vi "Process.vi"(8 "error in":errorcluster, 11 "Qbus in":refnum<class "Qbus.lvclass">) -> (0 "error out":errorcluster)   [LabVIEW 2021, in "AnalogGenerationProcess.lvlib"]
uses:
  AnalogGenerationProcess.lvlib
  <vilib>/addons/Qbus/Qbus.lvclass
  controls/state.ctl
  controls/generation status.ctl
  <vilib>/addons/_NISVFA/_Generation/Signal Generation/SV Signal/SV Signal.lvclass
  controls/analog generation settings.ctl
  controls/analog output settings.ctl
  controls/terminal configuration.ctl
  controls/signal settings.ctl
  controls/signal type.ctl
  shared/controls/digital output level units.ctl
  controls/sine wave properties.ctl
  <vilib>/addons/_NISVFA/_Generation/Signal Generation/SV Signal/sv_System Timing Model.ctl
  <vilib>/DAQmx/write.llb/DAQmx Write (Analog 1D Wfm NChan NSamp).vi
  <vilib>/addons/_NISVFA/_Generation/Signal Generation/SV Sinusoid/SV Sinusoid.lvclass
  C:/Program Files/National Instruments/LabVIEW 2021/vi.lib/addons/_NISVFA/_Generation/Signal Generation/SV Signal/SV Signal.lvclass
  <vilib>/addons/_NISVFA/_Generation/Signal Generation/SV Sinusoid/Configure Sine.vi
  <vilib>/addons/_NISVFA/_Generation/Signal Generation/SV Signal/Write Sample Rate.vi
  <vilib>/addons/_NISVFA/_Generation/Signal Generation/SV Signal/Write System Timing Model.vi
  <vilib>/addons/_NISVFA/_Generation/Signal Generation/SV Signal/Write Ramp Parameters.vi
  <vilib>/DAQmx/miscellaneous.llb/DAQmx Fill In Error Info.vi
  subVIs/utility/AudioGenUtility.lvlib
  shared/logger process/EventLoggerProcess.lvlib
  controls/AudioGenTypeDefs.lvlib
  shared/controls/audio controls.lvlib
  C:/Program Files/National Instruments/LabVIEW 2021/vi.lib/addons/_NISVFA/_Generation/Signal Generation/SV Function/SV Function.lvclass
  C:/Program Files/National Instruments/LabVIEW 2021/vi.lib/addons/_NISVFA/_Generation/Signal Generation/SV Sinusoid/SV Sinusoid.lvclass
  <vilib>/addons/_NISVFA/_Generation/Signal Generation/SV Multitone/SV Multitone.lvclass
  C:/Program Files/National Instruments/LabVIEW 2021/vi.lib/addons/_NISVFA/_Generation/Signal Generation/SV Multitone/SV Multitone.lvclass
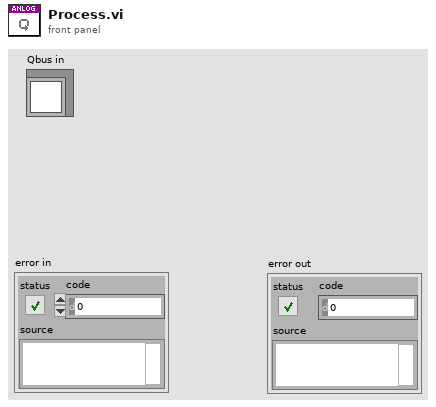
[diagram p1: front panel]
types:
  T1 = typedef "AnalogGenerationProcess.lvlib/state.ctl" = cluster{"DAQmx task":refnum<k21>, "status":T2, "signals":refnum<class "SV Signal.lvclass">[], "number of channels":u32}
  T2 = typedef "AudioGenTypeDefs.lvlib/generation status.ctl" = enum16{"Idle", "Committed", "Active"}
  T3 = typedef "AudioGenTypeDefs.lvlib/analog generation settings.ctl" = cluster{"channel list":string, "output settings":T4, "signal settings":T6}
  T4 = typedef "AudioGenTypeDefs.lvlib/analog output settings.ctl" = cluster{"output rate":dbl, "range":dbl, "terminal configuration":T5, "output impedance":dbl, "common mode offset":dbl, "pure tone mode":bool}
  T5 = typedef "AudioGenTypeDefs.lvlib/terminal configuration.ctl" = enum32{"Default", "RSE", "Differential", "Pseudodifferential"}
  T6 = typedef "AudioGenTypeDefs.lvlib/signal settings.ctl" = cluster{"signal type":T7, "properties":string, "output level units":T8}
  T7 = typedef "AudioGenTypeDefs.lvlib/signal type.ctl" = enum16{"Sine", "Dual Tone"}
  T8 = typedef "audio controls.lvlib/digital output level units.ctl" = enum32{"% FS", "dBFS", "V"}
  T9 = cluster{"profile":enum16{"Linear", "Half cosine"}, "durations [s]":cluster{"ramp-up":dbl, "transition":dbl, "ramp-down":dbl}}
  T10 = typedef "AudioGenTypeDefs.lvlib/sine wave properties.ctl" = cluster{"frequency":dbl, "amplitude":dbl, "phase":dbl}[]
  T11 = typedef "AudioGenTypeDefs.lvlib/dual tone properties.ctl" = cluster{"IMD type":T12, "low frequency":dbl, "high frequency":dbl, "amplitude ratio":dbl, "ampltidue":dbl}
  T12 = typedef "AudioGenTypeDefs.lvlib/dual tone types.ctl" = enum32{"SMPTE 4:1", "DIN", "CCIF 11k-12k", "CCIF 19k-20k", "Custom"}
  T13 = typedef "SV Signal.lvclass/sv_System Timing Model.ctl" = i64
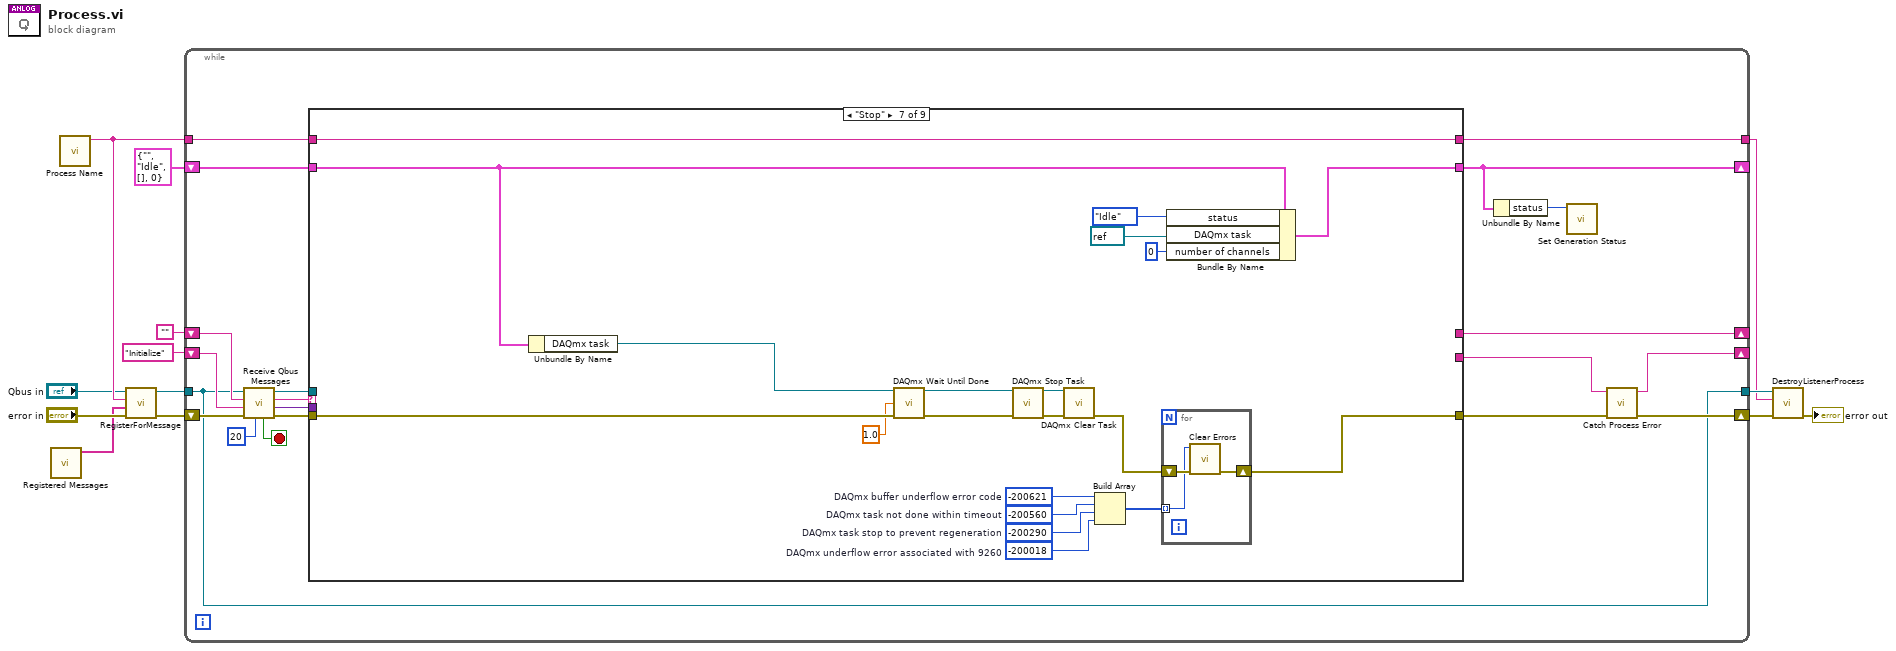
[diagram p0: block diagram]
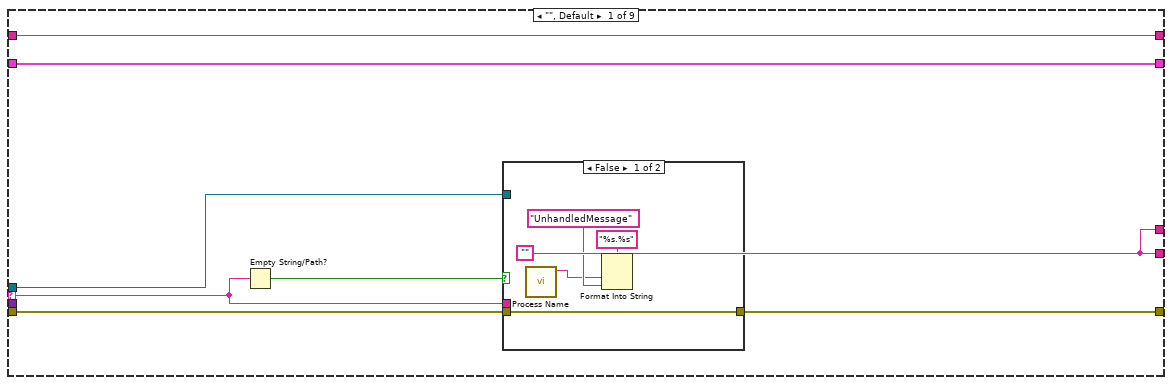
[diagram p2: hidden frame]
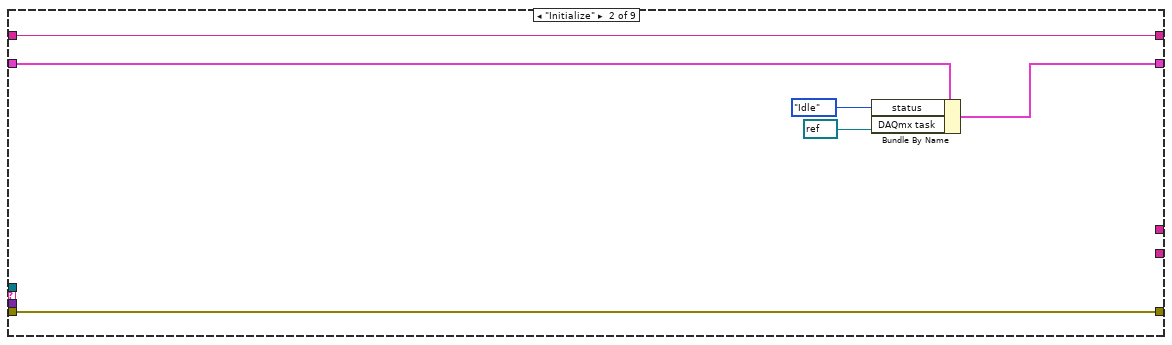
[diagram p4: hidden frame]
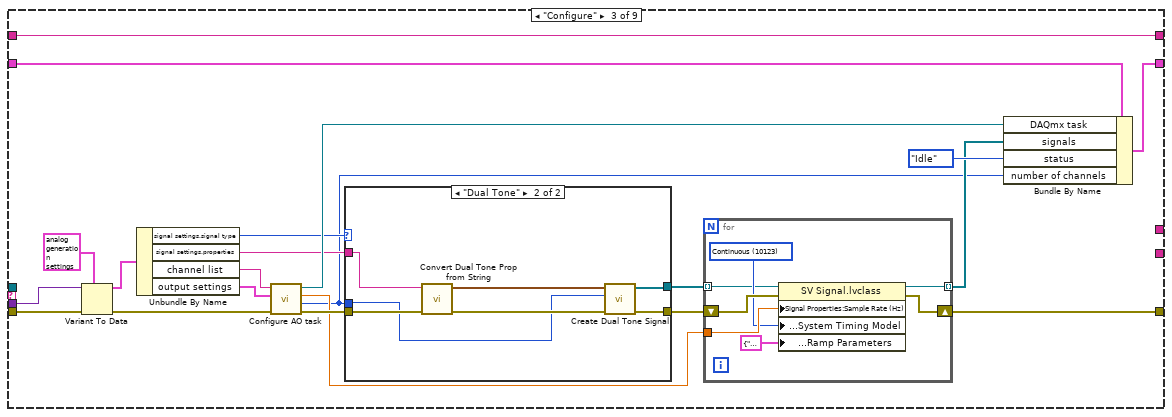
[diagram p5: hidden frame]
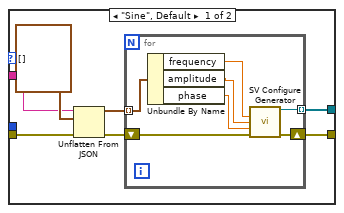
[diagram p6: hidden frame]
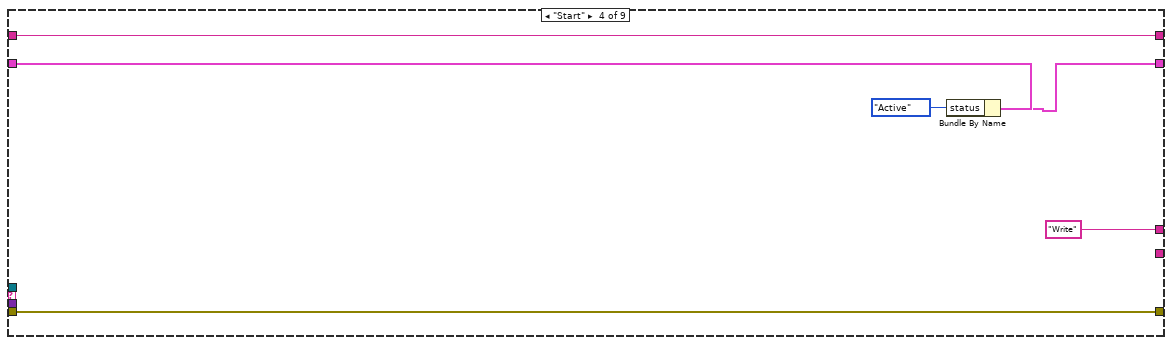
[diagram p7: hidden frame]
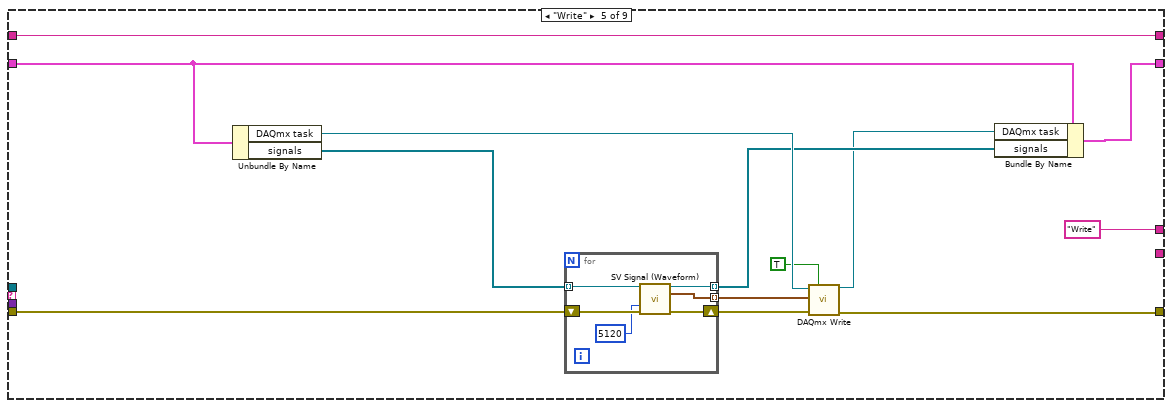
[diagram p8: hidden frame]
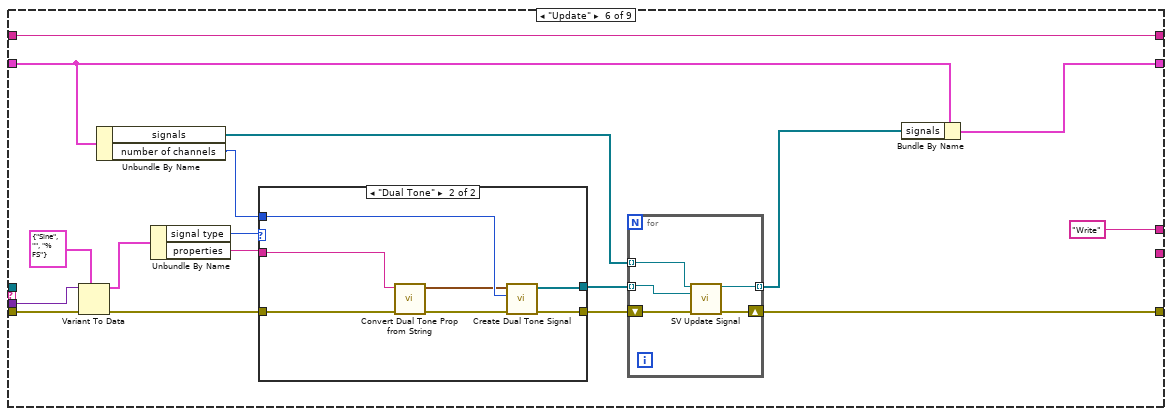
[diagram p9: hidden frame]
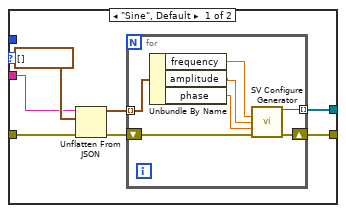
[diagram p10: hidden frame]
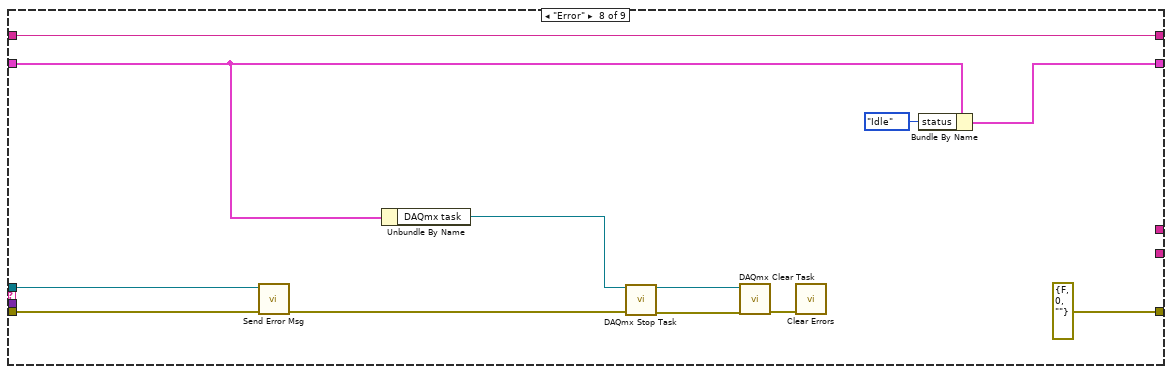
[diagram p11: hidden frame]
diagram:
  n1 = call "Registered Messages.vi"() -> ("registered messages"=w6:string[])  [unwired: 11 in]
  n2 = call "Process Name.vi"() -> ("process name"=w9:string)  [unwired: 11 in]
  n3 = call <vilib>:"RegisterForMessage.vi"("error in (no error)"="error in", "message names"=w6, "process name"=w9, "Qbus in"="Qbus in") -> ("error in (no error)"=w12:errorcluster, "Qbus out"=w13:refnum<class "Qbus.lvclass">)  [unwired: 6 in]
  n4 = while {
    shift-right: [w20] -> _
    shift-left: "" -> [w32]
    tunnel: w13 -> [w16]
    tunnel: w9 -> [w18]
    tunnel: [w16] -> w4
    tunnel: [w22] -> w2
    shift-right: [w26] -> _
    shift-left: "Initialize" -> [w28]
    shift-right: [w27] -> w5
    shift-left: w12 -> [w25]
    shift-right: [w15] -> _
    shift-left: T1 {"DAQmx task"="", "status"=enum."Idle", "signals"=[], "number of channels"=0} ("state") -> [w17]
    stop <- w33 stop-if-true
    n5 = call "Receive Qbus Messages.vi"("timeout(ms)"=20 ("milliseconds to wait"), "error in (no error)"=w25, "priority action"=w28, "default action"=w32, "Qbus in"=w16) -> ("error out"=w31:errorcluster, "message value"=w29:variant, "action"=w24:string, "Qbus out"=w30:refnum<class "Qbus.lvclass">, "exit"=w33:bool)  [unwired: 2 in]
    n6 = case shown="\"Stop\"" w24 {
      selector: w24 -> [w38 _ _ _ _ _ _ _ _]
      tunnel: w31 -> [w40 w52 w64 w107 w119 w139 w188 w203 w207]
      tunnel: w30 -> [w36 _ _ _ _ _ _ w202 _]
      tunnel: [w39 w52 w68 w107 w115 w129 w176 errorcluster {"status"=FALSE, "code"=0, "source"=""} ("error out") w207] -> w19
      tunnel: w29 -> [_ _ w65 _ _ w138 _ _ _]
      tunnel: [w41 w51 w73 w106 w120 w143 w189 w204 w206] -> w22
      tunnel: w18 -> [w41 w51 w73 w106 w120 w143 w189 w204 w206]
      tunnel: [w35 _ _ _ _ _ _ _ _] -> w21
      tunnel: [w35 _ _ "Write" "Write" "Write" _ _ _] -> w20
      tunnel: w17 -> [w34 w50 w72 w105 w111 w142 w184 w195 w205]
      tunnel: [w34 w49 w71 w103 w110 w141 w183 w194 w205] -> w15
      frame "", Default {
        w35 = ""
        n7 = Empty String/Path?(string/path=w38) -> (empty?=w37:bool)
        n8 = case shown="False" w37 {
          tunnel: [w42 w46] -> w39
          tunnel: w40 -> [w42 w46]
          tunnel: w38 -> [_ _]
          tunnel: w36 -> [_ _]
          frame False {
            n9 = call "Process Name.vi"() -> ("process name"=w43:string)  [unwired: 11 in]
            n10 = Format Into String(format string="%s.%s", w43, "UnhandledMessage" ("ProcessName")) -> ()  [unwired: 2 in, 2 out]
          }
          frame True {
          }
        }
      }
      frame "Initialize" {
        n11 = Bundle By Name(cluster=w50, "status"=enum16{"Idle", "Committed", "Active"}."Idle", "DAQmx task"=refnum<k21> refnum) -> (w49:T1)
      }
      frame "Configure" {
        n12 = Variant To Data(error in=w64, type=T3 {"channel list"="", "output settings"={"output rate"=0.0, "range"=0.0, "terminal configuration"=enum."Pseudodifferential", "output impedance"=0.0, "common mode offset"=0.0, "pure tone mode"=FALSE}, "signal settings"={"signal type"=enum."Sine", "properties"="", "output level units"=enum."% FS"}} ("analog generation"), Variant=w65) -> (data=w62:T3, error out=w61:errorcluster)
        n13 = Unbundle By Name(w62) -> ("signal settings.signal type"=w60:T7, "signal settings.properties"=w59:string, "channel list"=w58:string, "output settings"=w57:T4)
        n14 = call "Configure AO task.vi"("error in (no error)"=w61, "analog generation"=w57, "physical channels"=w58) -> ("error out"=w70:errorcluster, "number of channels"=w53:u32, "actual sample rate"=w67:dbl, "task out"=w66:refnum<k21>)  [unwired: 5 in]
        n15 = case shown="\"Dual Tone\"" w60 {
          tunnel: w70 -> [w85 w101]
          tunnel: [w87 w96] -> w55
          tunnel: [w86 w99] -> w69
          tunnel: w59 -> [w82 w100]
          tunnel: w53 -> [_ w95]
          frame "Sine", Default {
            n16 = Unflatten From JSON(JSON string=w82, type and defaults=T10 [] ("sine wave properties"), error in (no error)=w85) -> (value=w81:T10, error out=w84:errorcluster)  [unwired: 4 in]
            n17 = for {
              tunnel: [w94] -> w87 mode=indexing
              shift-right: [w93] -> w86
              shift-left: w84 -> [w92]
              tunnel: w81 -> [w91] mode=indexing
              n18 = Unbundle By Name(w91) -> ("frequency"=w90:dbl, "amplitude"=w89:dbl, "phase"=w88:dbl)
              n19 = call-poly <vilib>:"SV Configure Generator.vi"("frequency (Hz)"=w90, "amplitude"=w89, "phase (deg)"=w88, "error in (no error)"=w92) -> ("signal configuration"=w94:refnum<class "SV Sinusoid.lvclass">, "error out"=w93:errorcluster)  [unwired: 10 in]
            }
          }
          frame "Dual Tone" {
            n20 = call "Convert Dual Tone Prop from String.vi"("error in (no error)"=w101, "dual tone properties"=w100) -> ("error out"=w98:errorcluster, "dual tone properties"=w97:T11)  [unwired: 8 in]
            n21 = call "Create Dual Tone Signal.vi"("error in (no error)"=w98, "number of channels"=w95, "dual tone properties"=w97) -> ("error out"=w99:errorcluster, "signals"=w96:refnum<class "SV Multitone.lvclass">[])  [unwired: 7 in]
          }
        }
        n22 = for {
          tunnel: w67 -> [w78]
          shift-right: [w79] -> w68
          shift-left: w69 -> [w80]
          tunnel: w55 -> [w75] mode=indexing
          tunnel: [w74] -> w54 mode=indexing
          w77 = T13 10123 items=["Finite"=10178, "-"=-1, "Continuous"=10123, "-"=-2, "Settled"=110123, "Averaged"=210123, "Discrete Sweep"=310123, "Continuous Sweep"=410123] ("System Timing Model")
          n23 = property class="SV Signal.lvclass"(reference=w75, error in=w80, "Signal Properties:Sample Rate (Hz)"=w78, "Signal Properties:System Timing Model"=w77, "Signal Properties:Ramps:Ramp Parameters"=T9 {"profile"=enum."Half cosine", "durations [s]"={"ramp-up"=0.01, "transition"=0.01, "ramp-down"=0.01}} ("Ramp Parameters:All Elements")) -> (reference out=w74:refnum<class "SV Signal.lvclass">, error out=w79:errorcluster)
        }
        n24 = Bundle By Name(cluster=w72, "DAQmx task"=w66, "signals"=w54, "status"=generation_status."Idle", "number of channels"=w53) -> (w71:T1)
      }
      frame "Start" {
        n25 = Bundle By Name(cluster=w105, "status"=enum16{"Idle", "Committed", "Active"}."Active") -> (w103:T1)
      }
      frame "Write" {
        n26 = Unbundle By Name(w111) -> ("DAQmx task"=w116:refnum<k21>, "signals"=w118:refnum<class "SV Signal.lvclass">[])
        n27 = for {
          tunnel: w118 -> [w125] mode=indexing
          tunnel: [w122] -> w113 mode=indexing
          shift-right: [w124] -> w117
          shift-left: w119 -> [w126]
          tunnel: [w121] -> w108 mode=indexing
          n28 = call-dynamic "SV Signal (Waveform).vi"("signal configuration"=w125, "samples"=5120, "error in (no error)"=w126) -> ("signal configuration"=w122:refnum<class "SV Signal.lvclass">, "output waveform"=w121:waveform(dbl), "error out"=w124:errorcluster)  [unwired: 7 in, 3 out]
        }
        n29 = call-poly <vilib>:"DAQmx Write.vi"("task/channels in"=w116, "auto start"=TRUE, "data"=w108, "error in"=w117) -> ("task out"=w112:refnum<k21>, "error out"=w115:errorcluster)  [unwired: 9 in, 1 out]
        n30 = Bundle By Name(cluster=w111, "DAQmx task"=w112, "signals"=w113) -> (w110:T1)
      }
      frame "Update" {
        n31 = Variant To Data(error in=w139, type=T6 {"signal type"=enum."Sine", "properties"="", "output level units"=enum."% FS"} ("signal settings"), Variant=w138) -> (data=w137:T6, error out=w135:errorcluster)
        n32 = Unbundle By Name(w142) -> ("signals"=w132:refnum<class "SV Signal.lvclass">[], "number of channels"=w127:u32)
        n33 = Unbundle By Name(w137) -> ("signal type"=w134:T7, "properties"=w133:string)
        n34 = case shown="\"Dual Tone\"" w134 {
          tunnel: w135 -> [w153 w166]
          tunnel: [w155 w167] -> w131
          tunnel: [w154 w169] -> w130
          tunnel: w133 -> [w150 w163]
          tunnel: w127 -> [_ w168]
          frame "Sine", Default {
            n35 = Unflatten From JSON(JSON string=w150, type and defaults=T10 [] ("sine wave properties"), error in (no error)=w153) -> (value=w149:T10, error out=w152:errorcluster)  [unwired: 4 in]
            n36 = for {
              tunnel: [w162] -> w155 mode=indexing
              shift-right: [w161] -> w154
              shift-left: w152 -> [w160]
              tunnel: w149 -> [w159] mode=indexing
              n37 = Unbundle By Name(w159) -> ("frequency"=w158:dbl, "amplitude"=w157:dbl, "phase"=w156:dbl)
              n38 = call-poly <vilib>:"SV Configure Generator.vi"("frequency (Hz)"=w158, "amplitude"=w157, "phase (deg)"=w156, "error in (no error)"=w160) -> ("signal configuration"=w162:refnum<class "SV Sinusoid.lvclass">, "error out"=w161:errorcluster)  [unwired: 10 in]
            }
          }
          frame "Dual Tone" {
            n39 = call "Convert Dual Tone Prop from String.vi"("error in (no error)"=w166, "dual tone properties"=w163) -> ("error out"=w165:errorcluster, "dual tone properties"=w164:T11)  [unwired: 8 in]
            n40 = call "Create Dual Tone Signal.vi"("error in (no error)"=w165, "number of channels"=w168, "dual tone properties"=w164) -> ("error out"=w169:errorcluster, "signals"=w167:refnum<class "SV Multitone.lvclass">[])  [unwired: 7 in]
          }
        }
        n41 = for {
          tunnel: w132 -> [w146] mode=indexing
          tunnel: w131 -> [w147] mode=indexing
          shift-right: [w145] -> w129
          shift-left: w130 -> [w148]
          tunnel: [w144] -> w128 mode=indexing
          n42 = call-dynamic "SV Update Signal.vi"("current configuration"=w146, "new configuration"=w147, "error in (no error)"=w148) -> ("updated configuration"=w144:refnum<class "SV Signal.lvclass">, "error out"=w145:errorcluster)  [unwired: 11 in]
        }
        n43 = Bundle By Name(cluster=w142, "signals"=w128) -> (w141:T1)
      }
      frame "Stop" {
        w179 = -200018  # DAQmx underflow error associated with 9260
        w180 = -200290  # DAQmx task stop to prevent regeneration
        w181 = -200560  # DAQmx task not done within timeout
        w182 = -200621  # DAQmx buffer underflow error code
        n44 = Unbundle By Name(w184) -> ("DAQmx task"=w187:refnum<k21>)
        n45 = call <vilib>:"DAQmx Wait Until Done.vi"("task/channels in"=w187, "timeout (sec)"=1.0, "error in"=w188) -> ("task out"=w186:refnum<k21>, "error out"=w177:errorcluster)  [unwired: 11 in]
        n46 = call <vilib>:"DAQmx Stop Task.vi"("task/channels in"=w186, "error in"=w177) -> ("task out"=w174:refnum<k21>, "error out"=w173:errorcluster)  [unwired: 12 in]
        n47 = call <vilib>:"DAQmx Clear Task.vi"("task in"=w174, "error in"=w173) -> ("error out"=w172:errorcluster)  [unwired: 13 in]
        n48 = Build Array(w182, w181, w180, w179) -> (w178:i32[])
        n49 = for {
          shift-right: [w191] -> w176
          shift-left: w172 -> [w192]
          tunnel: w178 -> [w190] mode=indexing
          n50 = call <vilib>:"Clear Errors.vi"("error in (no error)"=w192, "specific error code to clear (0: all)"=w190) -> ("error out"=w191:errorcluster)  [unwired: 4 in, 1 out]
        }
        n51 = Bundle By Name(cluster=w184, "status"=generation_status."Idle", "DAQmx task"=refnum<k21> refnum, "number of channels"=u32 0) -> (w183:T1)
      }
      frame "Error" {
        n52 = call "Send Error Msg.vi"("error in"=w203, "Qbus in"=w202) -> ("error out"=w200:errorcluster)  [unwired: 8 in, 1 out]
        n53 = Unbundle By Name(w195) -> ("DAQmx task"=w199:refnum<k21>)
        n54 = call <vilib>:"DAQmx Stop Task.vi"("task/channels in"=w199, "error in"=w200) -> ("task out"=w198:refnum<k21>, "error out"=w197:errorcluster)  [unwired: 12 in]
        n55 = call <vilib>:"DAQmx Clear Task.vi"("task in"=w198, "error in"=w197) -> ("error out"=w196:errorcluster)  [unwired: 13 in]
        n56 = call <vilib>:"Clear Errors.vi"("error in (no error)"=w196) -> ()  [unwired: 5 in, 2 out]
        n57 = Bundle By Name(cluster=w195, "status"=generation_status."Idle") -> (w194:T1)
      }
      frame "Exit" {
      }
    }
    n58 = Unbundle By Name(w15) -> ("status"=w14:T2)
    n59 = call "Set Generation Status.vi"("status"=w14) -> ()  [unwired: 10 in, 1 out]
    n60 = call "Catch Process Error.vi"("error in (no error)"=w19, "priority action"=w21) -> ("error out"=w27:errorcluster, "priority action"=w26:string)  [unwired: 8 in]
  }
  n61 = call <vilib>:"DestroyListenerProcess.vi"("error in (no error)"=w5, "process name"=w2, "Qbus in"=w4) -> ("error in (no error)"=→"error out":errorcluster)  [unwired: 7 in, 1 out]
